vi "All Vis.vi"   [LabVIEW 2012, in "Scripting Tools.lvlib"]
uses:
  Scripting Tools.lvlib
  Public/Create LVObject references/Polymorphs/Generic reference.vi
  Primatives/Array/Create Replace Array 1D Multiple.vi
  Primatives/Array/Create Insert into Array 1D Multiple.vi
  Primatives/Array/Create Delete Array nD Single.vi
  Primatives/Array/Create Array Subset Multiple.vi
  Primatives/Array/Create Build Array Single.vi
  Primatives/Vi Server/Polymorphs/Create Property Node(class name).vi
  XNode Support/XNode Support.lvlib
  Public/Create Free Text Label Polymorphs/Create a free text label on FP.vi
  XNode Support/Find term type by ID_Terminal.vi
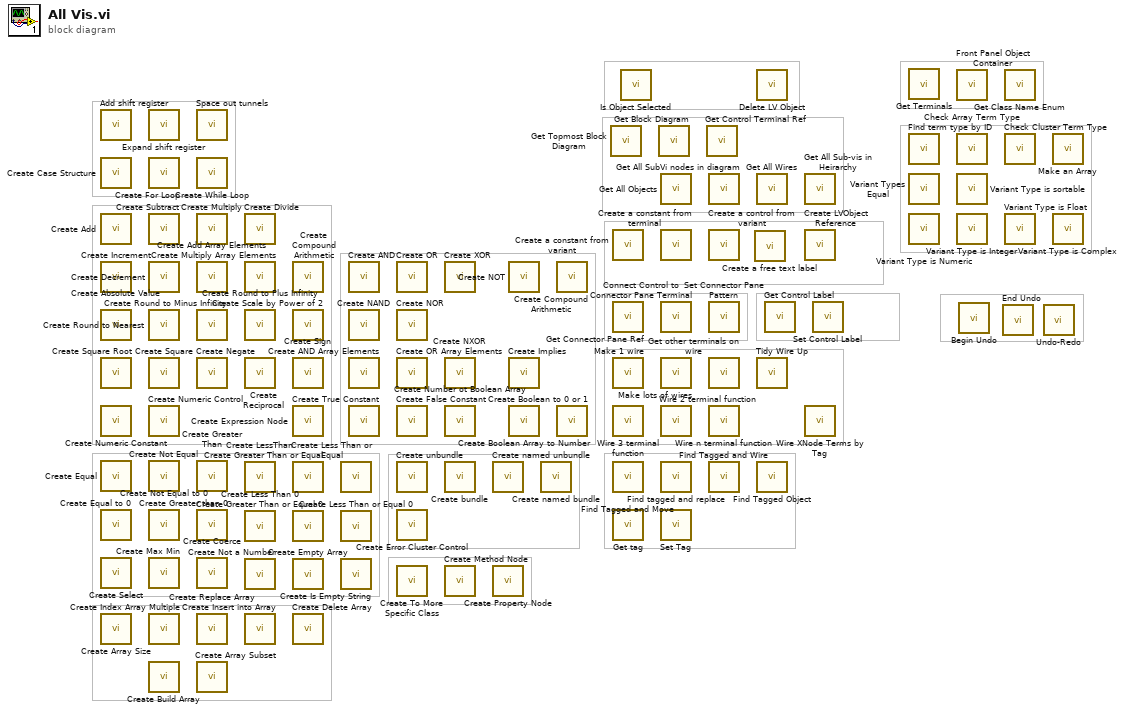
[diagram p0: block diagram]
diagram:
  n1 = call "Add shift register.vi"() -> ()  [unwired: 9 in, 7 out]
  n2 = call "Create Case Structure.vi"() -> ()  [unwired: 11 in, 5 out]
  n3 = call "Create Add.vi"() -> ()  [unwired: 9 in, 3 out]
  n4 = call "Create Increment.vi"() -> ()  [unwired: 9 in, 3 out]
  n5 = call "Create Absolute Value.vi"() -> ()  [unwired: 9 in, 3 out]
  n6 = call "Create Square Root.vi"() -> ()  [unwired: 9 in, 3 out]
  n7 = call "Create Numeric Constant.vi"() -> ()  [unwired: 9 in, 3 out]
  n8 = call "Create Equal.vi"() -> ()  [unwired: 9 in, 3 out]
  n9 = call "Create Equal to 0.vi"() -> ()  [unwired: 9 in, 3 out]
  n10 = call "Create Select.vi"() -> ()  [unwired: 9 in, 3 out]
  n11 = call "Create Array Size.vi"() -> ()  [unwired: 9 in, 3 out]
  n12 = call "Expand shift register.vi"() -> ()  [unwired: 8 in, 4 out]
  n13 = call "Create For Loop.vi"() -> ()  [unwired: 10 in, 6 out]
  n14 = call "Create Subtract.vi"() -> ()  [unwired: 9 in, 3 out]
  n15 = call "Create Decrement.vi"() -> ()  [unwired: 9 in, 3 out]
  n16 = call "Create Round to Nearest.vi"() -> ()  [unwired: 9 in, 3 out]
  n17 = call "Create Square.vi"() -> ()  [unwired: 9 in, 3 out]
  n18 = call "Create Numeric Control.vi"() -> ()  [unwired: 9 in, 3 out]
  n19 = call "Create Not Equal.vi"() -> ()  [unwired: 9 in, 3 out]
  n20 = call "Create Not Equal to 0.vi"() -> ()  [unwired: 9 in, 3 out]
  n21 = call "Create Max Min.vi"() -> ()  [unwired: 8 in, 4 out]
  n22 = call "Create Index Array Multiple.vi"() -> ()  [unwired: 9 in, 3 out]
  n23 = call-poly "Create Build Array.vi"() -> ()  [unwired: 9 in, 3 out]
  n24 = call "Space out tunnels.vi"() -> ()  [unwired: 8 in, 4 out]
  n25 = call "Create While Loop.vi"() -> ()  [unwired: 11 in, 5 out]
  n26 = call "Create Multiply.vi"() -> ()  [unwired: 9 in, 3 out]
  n27 = call "Create Add Array Elements.vi"() -> ()  [unwired: 9 in, 3 out]
  n28 = call "Create Round to Minus Infinity.vi"() -> ()  [unwired: 9 in, 3 out]
  n29 = call "Create Negate.vi"() -> ()  [unwired: 9 in, 3 out]
  n30 = call "Create Greater Than.vi"() -> ()  [unwired: 9 in, 3 out]
  n31 = call "Create Greater than 0.vi"() -> ()  [unwired: 9 in, 3 out]
  n32 = call "Create Coerce.vi"() -> ()  [unwired: 8 in, 4 out]
  n33 = call-poly "Create Replace Array.vi"() -> ()  [unwired: 9 in, 3 out]
  n34 = call-poly "Create Array Subset.vi"() -> ()  [unwired: 9 in, 3 out]
  n35 = call "Create Divide.vi"() -> ()  [unwired: 9 in, 3 out]
  n36 = call "Create Multiply Array Elements.vi"() -> ()  [unwired: 9 in, 3 out]
  n37 = call "Create Round to Plus Infinity.vi"() -> ()  [unwired: 9 in, 3 out]
  n38 = call "Create Reciprocal.vi"() -> ()  [unwired: 9 in, 3 out]
  n39 = call "Create LessThan.vi"() -> ()  [unwired: 9 in, 3 out]
  n40 = call "Create Less Than 0.vi"() -> ()  [unwired: 9 in, 3 out]
  n41 = call "Create Not a Number.vi"() -> ()  [unwired: 9 in, 3 out]
  n42 = call-poly "Create Insert into Array.vi"() -> ()  [unwired: 9 in, 3 out]
  n43 = call "Create Compound Arithmetic.vi"() -> ()  [unwired: 9 in, 3 out]
  n44 = call "Create Scale by Power of 2.vi"() -> ()  [unwired: 9 in, 3 out]
  n45 = call "Create Sign.vi"() -> ()  [unwired: 9 in, 3 out]
  n46 = call "Create Expression Node.vi"() -> ()  [unwired: 9 in, 3 out]
  n47 = call "Create Greater Than or Equal.vi"() -> ()  [unwired: 9 in, 3 out]
  n48 = call "Create Greater Than or Equal 0.vi"() -> ()  [unwired: 9 in, 3 out]
  n49 = call "Create Empty Array.vi"() -> ()  [unwired: 9 in, 3 out]
  n50 = call-poly "Create Delete Array.vi"() -> ()  [unwired: 8 in, 4 out]
  n51 = call "Create Less Than or Equal.vi"() -> ()  [unwired: 9 in, 3 out]
  n52 = call "Create Less Than or Equal 0.vi"() -> ()  [unwired: 9 in, 3 out]
  n53 = call "Create Is Empty String.vi"() -> ()  [unwired: 9 in, 3 out]
  n54 = call "Create AND.vi"() -> ()  [unwired: 9 in, 3 out]
  n55 = call "Create NAND.vi"() -> ()  [unwired: 9 in, 3 out]
  n56 = call "Create AND Array Elements.vi"() -> ()  [unwired: 9 in, 3 out]
  n57 = call "Create True Constant.vi"() -> ()  [unwired: 9 in, 3 out]
  n58 = call "Create OR.vi"() -> ()  [unwired: 9 in, 3 out]
  n59 = call "Create NOR.vi"() -> ()  [unwired: 9 in, 3 out]
  n60 = call "Create OR Array Elements.vi"() -> ()  [unwired: 9 in, 3 out]
  n61 = call "Create False Constant.vi"() -> ()  [unwired: 9 in, 3 out]
  n62 = call "Create unbundle.vi"() -> ()  [unwired: 9 in, 3 out]
  n63 = call "Create Error Cluster Control.vi"() -> ()  [unwired: 9 in, 3 out]
  n64 = call "Create To More Specific Class.vi"() -> ()  [unwired: 8 in, 4 out]
  n65 = call "Create XOR.vi"() -> ()  [unwired: 9 in, 3 out]
  n66 = call "Create NXOR.vi"() -> ()  [unwired: 9 in, 3 out]
  n67 = call "Create Number ot Boolean Array.vi"() -> ()  [unwired: 9 in, 3 out]
  n68 = call "Create bundle.vi"() -> ()  [unwired: 9 in, 3 out]
  n69 = call "Create Method Node.vi"() -> ()  [unwired: 11 in, 5 out]
  n70 = call "Create named unbundle.vi"() -> ()  [unwired: 9 in, 3 out]
  n71 = call-poly "Create Property Node.vi"() -> ()  [unwired: 11 in, 5 out]
  n72 = call "Create NOT.vi"() -> ()  [unwired: 9 in, 3 out]
  n73 = call "Create Implies.vi"() -> ()  [unwired: 9 in, 3 out]
  n74 = call "Create Boolean Array to Number.vi"() -> ()  [unwired: 9 in, 3 out]
  n75 = call "Create named bundle.vi"() -> ()  [unwired: 10 in, 2 out]
  n76 = call "Create Compound Arithmetic.vi"() -> ()  [unwired: 9 in, 3 out]
  n77 = call "Create Boolean to 0 or 1.vi"() -> ()  [unwired: 9 in, 3 out]
  n78 = call "Get Topmost Block Diagram.vi"() -> ()  [unwired: 9 in, 3 out]
  n79 = call "Create a constant from variant.vi"() -> ()  [unwired: 9 in, 3 out]
  n80 = call "Get Connector Pane Ref.vi"() -> ()  [unwired: 2 in, 3 out]
  n81 = call "Make 1 wire.vi"() -> ()  [unwired: 9 in, 3 out]
  n82 = call "Wire 3 terminal function.vi"() -> ()  [unwired: 9 in, 3 out]
  n83 = call "Find Tagged and Move.vi"() -> ()  [unwired: 10 in, 2 out]
  n84 = call "Get tag.vi"() -> ()  [unwired: 7 in, 5 out]
  n85 = call "Is Object Selected.vi"() -> ()  [unwired: 10 in, 2 out]
  n86 = call "Get Block Diagram.vi"() -> ()  [unwired: 2 in, 3 out]
  n87 = call "Get All Objects.vi"() -> ()  [unwired: 2 in, 3 out]
  n88 = call "Create a constant from terminal.vi"() -> ()  [unwired: 9 in, 3 out]
  n89 = call "Connect Control to Connector Pane Terminal.vi"() -> ()  [unwired: 5 in, 2 out]
  n90 = call "Make lots of wires.vi"() -> ()  [unwired: 10 in, 2 out]
  n91 = call "Wire 2 terminal function.vi"() -> ()  [unwired: 9 in, 3 out]
  n92 = call "Find tagged and replace.vi"() -> ()  [unwired: 10 in, 2 out]
  n93 = call "Set Tag.vi"() -> ()  [unwired: 9 in, 3 out]
  n94 = call "Get Control Terminal Ref.vi"() -> ()  [unwired: 2 in, 3 out]
  n95 = call "Get All SubVi nodes in diagram.vi"() -> ()  [unwired: 7 in, 5 out]
  n96 = call "Create a control from variant.vi"() -> ()  [unwired: 9 in, 3 out]
  n97 = call "Set Connector Pane Pattern.vi"() -> ()  [unwired: 6 in, 3 out]
  n98 = call "Get other terminals on wire.vi"() -> ()  [unwired: 8 in, 4 out]
  n99 = call "Wire n terminal function.vi"() -> ()  [unwired: 9 in, 3 out]
  n100 = call "Find Tagged and Wire.vi"() -> ()  [unwired: 10 in, 2 out]
  n101 = call-poly "Create a free text label.vi"() -> ()  [unwired: 10 in, 2 out]
  n102 = call "Delete LV Object.vi"() -> ()  [unwired: 10 in, 1 out]
  n103 = call "Get All Wires.vi"() -> ()  [unwired: 2 in, 3 out]
  n104 = call "Tidy Wire Up.vi"() -> ()  [unwired: 10 in, 2 out]
  n105 = call "Find Tagged Object.vi"() -> ()  [unwired: 9 in, 3 out]
  n106 = call "Get Control Label.vi"() -> ()  [unwired: 2 in, 3 out]
  n107 = call "Get All Sub-vis in Heirarchy.vi"() -> ()  [unwired: 7 in, 5 out]
  n108 = call-poly "Create LVObject Reference.vi"() -> ()  [unwired: 1 out]
  n109 = call "Wire XNode Terms by Tag.vi"() -> ()  [unwired: 11 in, 1 out]
  n110 = call "Set Control Label.vi"() -> ()  [unwired: 3 in, 2 out]
  n111 = call "Get Terminals.vi"() -> ()  [unwired: 9 in, 3 out]
  n112 = call-poly "Find term type by ID.vi"() -> ()  [unwired: 7 in, 5 out]
  n113 = call "Variant Types Equal.vi"() -> ()  [unwired: 10 in, 2 out]
  n114 = call "Variant Type is Numeric.vi"() -> ()  [unwired: 10 in, 2 out]
  n115 = call "Front Panel Object Container.vi"() -> ()  [unwired: 1 in]
  n116 = call "Check Array Term Type.vi"() -> ()  [unwired: 8 in, 4 out]
  n117 = call "Variant Type is sortable.vi"() -> ()  [unwired: 10 in, 2 out]
  n118 = call "Variant Type is Integer.vi"() -> ()  [unwired: 10 in, 2 out]
  n119 = call "Begin Undo.vi"() -> ()  [unwired: 10 in, 2 out]
  n120 = call "End Undo.vi"() -> ()  [unwired: 10 in, 2 out]
  n121 = call "Get Class Name Enum.vi"() -> ()  [unwired: 10 in, 2 out]
  n122 = call "Check Cluster Term Type.vi"() -> ()  [unwired: 9 in, 3 out]
  n123 = call "Variant Type is Float.vi"() -> ()  [unwired: 10 in, 2 out]
  n124 = call "Undo-Redo.vi"() -> ()  [unwired: 10 in, 2 out]
  n125 = call "Make an Array.vi"() -> ()  [unwired: 10 in, 2 out]
  n126 = call "Variant Type is Complex.vi"() -> ()  [unwired: 10 in, 2 out]
